vi "LoadCFG.vi"(8 "error in (no error)":errorcluster, 11 "object in":refnum<class "Configuration.lvclass">) -> (0 "error out":errorcluster, 2 "Success?":bool, 3 "object out":refnum<class "Configuration.lvclass">)   [LabVIEW 2021, in "Channel.lvlib" / "Configuration.lvclass"]
doc: "Loads the configuration"
uses:
  Configuration.lvclass
  Configuration.lvclass/Configuration.ctl
  <vilib>/Utility/config.llb/NI_LVConfig.lvlib
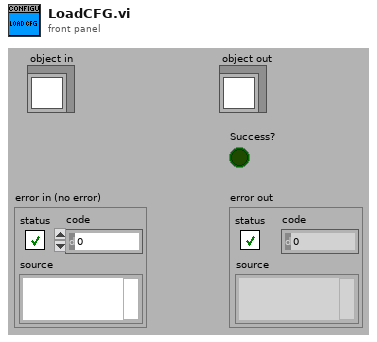
[diagram p1: front panel]
types:
  T1 = typedef "NI_LVConfig.lvlib/Config Data RefNum.ctl" = refnum<k1>
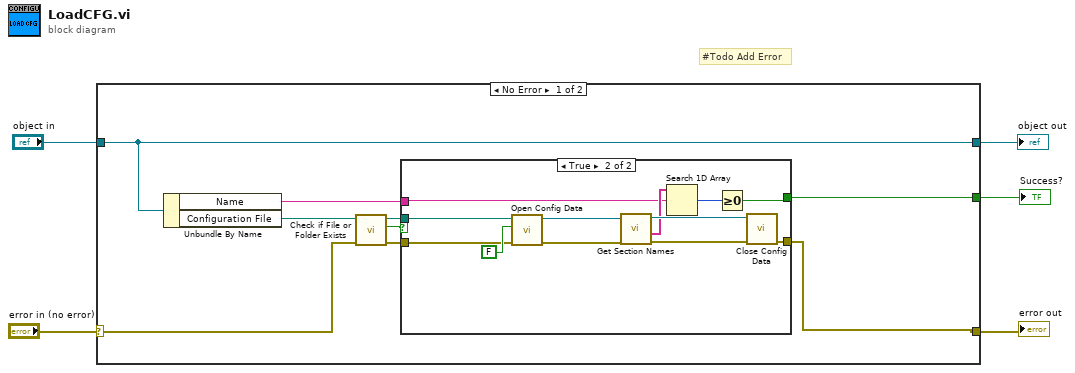
[diagram p0: block diagram]
diagram:
  # "#Todo Add Error"
  n1 = case shown="No Error" "error in (no error)" {
    selector: "error in (no error)" -> [w10 w30]
    tunnel: [w13 w30] -> w4
    tunnel: [w14 w29] -> w2
    tunnel: "object in" -> [w14 w29]
    tunnel: [w7 _] -> w1
    frame No Error {
      n2 = Unbundle By Name(w14) -> ("Name"=w12:string, "Configuration File"=w11:path)
      n3 = call <vilib>:"Check if File or Folder Exists.vi"("error in (no error)"=w10, "path"=w11) -> ("error out"=w9:errorcluster, "file or folder exists?"=w8:bool, "dup path"=w6:path)  [unwired: 7 in]
      n4 = case shown="True" w8 {
        selector: w8 -> [w15 _]
        tunnel: [w16 w23] -> w13
        tunnel: w12 -> [_ w19]
        tunnel: w9 -> [w16 w22]
        tunnel: [w15 w17] -> w7
        tunnel: w6 -> [_ w21]
        frame False {
        }
        frame True {
          n5 = call <vilib>:"Open Config Data.vi"("error in (no error)"=w22, "create file if necessary (T)"=FALSE, "configuration file path"=w21) -> ("error out"=w25:errorcluster, "refnum"=w28:T1)  [unwired: 6 in, 1 out]
          n6 = call <vilib>:"Get Section Names.vi"("error in (no error)"=w25, "refnum"=w28) -> ("error out"=w24:errorcluster, "section names"=w20:string[], "refnum out"=w27:T1)  [unwired: 7 in]
          n7 = Search 1D Array(1D array=w20, element=w19) -> (index of element=w18:i32)  [unwired: 1 in]
          n8 = Greater Or Equal To 0?(x=w18) -> (x >= 0?=w17:bool)
          n9 = call <vilib>:"Close Config Data.vi"("error in (no error)"=w24, "refnum"=w27) -> ("error out"=w23:errorcluster)  [unwired: 8 in, 1 out]
        }
      }
    }
    frame Error {
    }
  }
  "error out" <- w4
  "object out" <- w2
  "Success?" <- w1
